vi "Sample.vi"(8 "错误输入（无错误）":errorcluster, 9 "Device Info.开关":T1, 10 "双通道设备？":bool, 11 "VISA资源名称":refnum<visa-resource-name>) -> (0 "error out":errorcluster, 2 "Data Out":dbl[](array[numeric]) format="%.2f")   [LabVIEW 2026, in "UI-温度控制.lvlib" / "Acquisition.lvlib"]
uses:
  Acquisition.lvlib
  Supports/Device Info.ctl
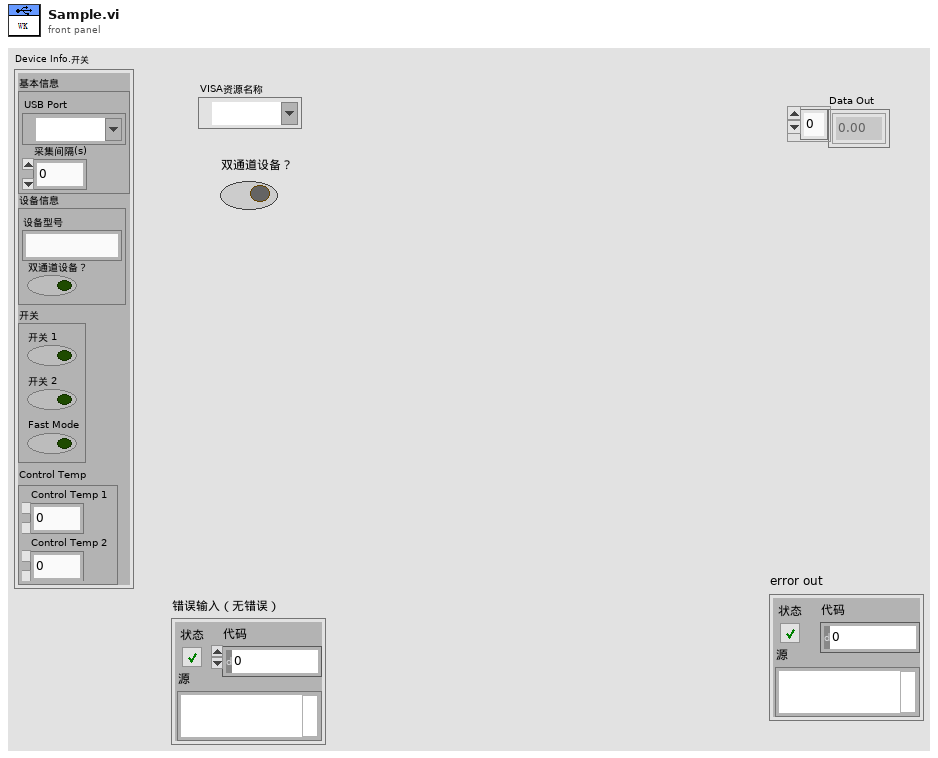
[diagram p1: front panel]
types:
  T1 = typedef "UI-温度控制.lvlib/Device Info.ctl" = cluster{"基本信息":cluster{"USB Port":refnum<visa-resource-name>, "采集间隔(s)":dbl}, "设备信息":cluster{"设备型号":string, "双通道设备？":bool}, "开关":cluster{"开关 1":bool, "开关 2":bool, "Fast Mode":bool}, "Control Temp":cluster{"Control Temp 1":dbl, "Control Temp 2":dbl}}
  T2 = cluster{"Control Temp 1":dbl, "Control Temp 2":dbl}
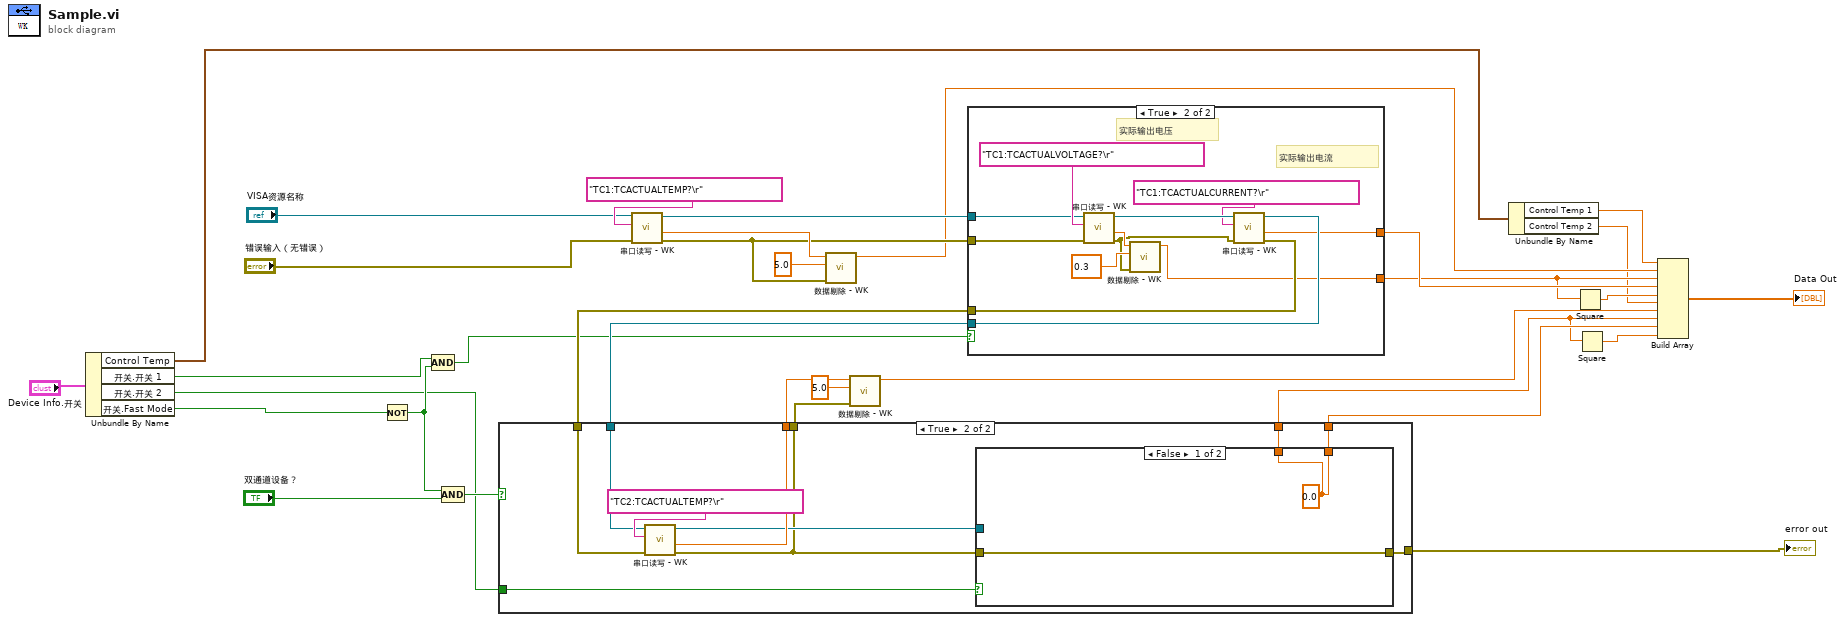
[diagram p0: block diagram]
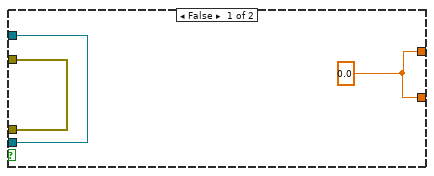
[diagram p2: hidden frame]
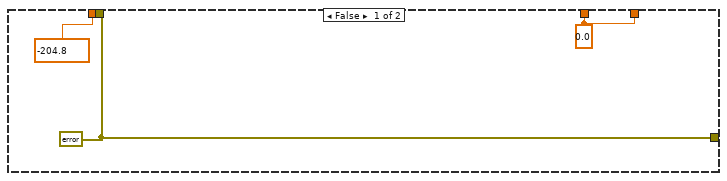
[diagram p3: hidden frame]
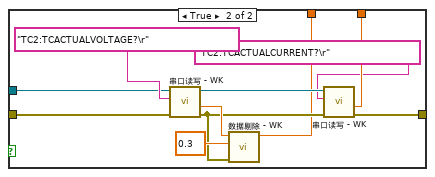
[diagram p4: hidden frame]
diagram:
  n1 = Unbundle By Name("Device Info.开关") -> ("Control Temp"=w3:T2, "开关.开关 1"=w14:bool, "开关.开关 2"=w8:bool, "开关.Fast Mode"=w13:bool)
  n2 = Not(x=w13) -> (.not. x?=w10:bool)
  n3 = Compound Arithmetic op=AND ("复合运算")(w14, w10) -> (w9:bool)
  n4 = Compound Arithmetic op=AND ("复合运算")(w10, "双通道设备？") -> (w11:bool)
  n5 = call "串口读写 - WK.vi"("错误输入（无错误）"="错误输入（无错误）", "写入设备"="TC1:TCACTUALTEMP?\r" ("写入缓冲区"), "VISA输入"="VISA资源名称") -> ("错误输出"=w24:errorcluster, "读取设备(n)"=w32:dbl, "VISA输出"=w25:refnum<visa-resource-name>)  [unwired: 5 in, 1 out]
  n6 = call "数据剔除 - WK.vi"("错误常量"=w24, "阈值"=5.0, "数据输入"=w32) -> ("数据输出"=w21:dbl)  [unwired: 8 in]
  n7 = case shown="True" w9 {
    tunnel: w25 -> [w36 w43]
    tunnel: w24 -> [w35 w42]
    tunnel: [w36 w40] -> w23
    tunnel: [w35 w39] -> w22
    tunnel: [w34 w38] -> w7
    tunnel: [w34 w37] -> w20
    frame False {
      w34 = 0.0
    }
    frame True {
      # "实际输出电流"
      # "实际输出电压"
      n8 = call "串口读写 - WK.vi"("错误输入（无错误）"=w42, "写入设备"="TC1:TCACTUALVOLTAGE?\r" ("写入缓冲区"), "VISA输入"=w43) -> ("错误输出"=w41:errorcluster, "读取设备(n)"=w44:dbl, "VISA输出"=w48:refnum<visa-resource-name>)  [unwired: 5 in, 1 out]
      n9 = call "数据剔除 - WK.vi"("错误常量"=w41, "阈值"=0.3, "数据输入"=w44) -> ("数据输出"=w38:dbl)  [unwired: 8 in]
      n10 = call "串口读写 - WK.vi"("错误输入（无错误）"=w41, "写入设备"="TC1:TCACTUALCURRENT?\r" ("写入缓冲区"), "VISA输入"=w48) -> ("错误输出"=w39:errorcluster, "读取设备(n)"=w37:dbl, "VISA输出"=w40:refnum<visa-resource-name>)  [unwired: 5 in, 1 out]
    }
  }
  n11 = case shown="True" w11 {
    tunnel: [-204.8 ("读取设备(n)") w60] -> w29
    tunnel: [w49 w56] -> w28
    tunnel: w23 -> [_ w59]
    tunnel: w22 -> [_ w58]
    tunnel: [w50 w55] -> w5
    tunnel: [w50 w54] -> w18
    tunnel: [w49 w53] -> w16
    tunnel: w8 -> [_ w52]
    frame False {
      w50 = 0.0 ("数据输出")
      w49 = errorcluster {"status"=FALSE, "code"=0, "source"=""} ("错误输出")
    }
    frame True {
      n12 = call "串口读写 - WK.vi"("错误输入（无错误）"=w58, "写入设备"="TC2:TCACTUALTEMP?\r" ("写入缓冲区"), "VISA输入"=w59) -> ("错误输出"=w56:errorcluster, "读取设备(n)"=w60:dbl, "VISA输出"=w57:refnum<visa-resource-name>)  [unwired: 5 in, 1 out]
      n13 = case shown="False" w52 {
        tunnel: w57 -> [_ w70]
        tunnel: w56 -> [w62 w69]
        tunnel: [w63 w67] -> w55
        tunnel: [w63 w66] -> w54
        tunnel: [w62 w65] -> w53
        frame False {
          w63 = 0.0
        }
        frame True {
          n14 = call "串口读写 - WK.vi"("错误输入（无错误）"=w69, "写入设备"="TC2:TCACTUALVOLTAGE?\r" ("写入缓冲区"), "VISA输入"=w70) -> ("错误输出"=w68:errorcluster, "读取设备(n)"=w74:dbl, "VISA输出"=w73:refnum<visa-resource-name>)  [unwired: 5 in, 1 out]
          n15 = call "数据剔除 - WK.vi"("错误常量"=w68, "阈值"=0.3, "数据输入"=w74) -> ("数据输出"=w67:dbl)  [unwired: 8 in]
          n16 = call "串口读写 - WK.vi"("错误输入（无错误）"=w68, "写入设备"="TC2:TCACTUALCURRENT?\r" ("写入缓冲区"), "VISA输入"=w73) -> ("错误输出"=w65:errorcluster, "读取设备(n)"=w66:dbl)  [unwired: 5 in, 2 out]
        }
      }
    }
  }
  "error out" <- w16
  n17 = call "数据剔除 - WK.vi"("错误常量"=w28, "阈值"=5.0, "数据输入"=w29) -> ("数据输出"=w19:dbl)  [unwired: 8 in]
  n18 = Unbundle By Name(w3) -> ("Control Temp 1"=w2:dbl, "Control Temp 2"=w1:dbl)
  n19 = Square(x=w7) -> (x^2=w6:dbl)
  n20 = Square(x=w5) -> (x^2=w4:dbl)
  n21 = Build Array(w2, w21, w7, w20, w6, w1, w19, w5, w18, w4) -> (→"Data Out":dbl[])
